vi "Rover_Planting_Commands.vi"(1 "X":dbl[](array[numeric]), 2 "Y":dbl[](array[numeric]), 3 "Seeds":bool[](array[boolean])) -> (0 "Commands":string[](array[string]), 4 "Expected":string[](array[string]), 5 "Count":i32)   [LabVIEW 2022]
doc: "Build line commands and exact acknowledgements from graph units. Does not move motors. One unit is 10 cm. Caller validates sizes and coordinate ranges."
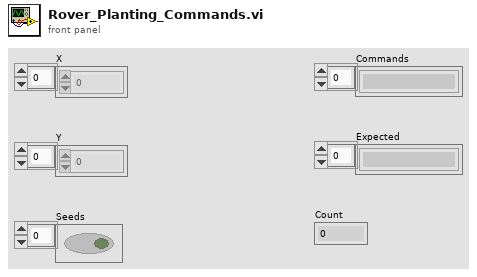
[diagram p1: front panel]
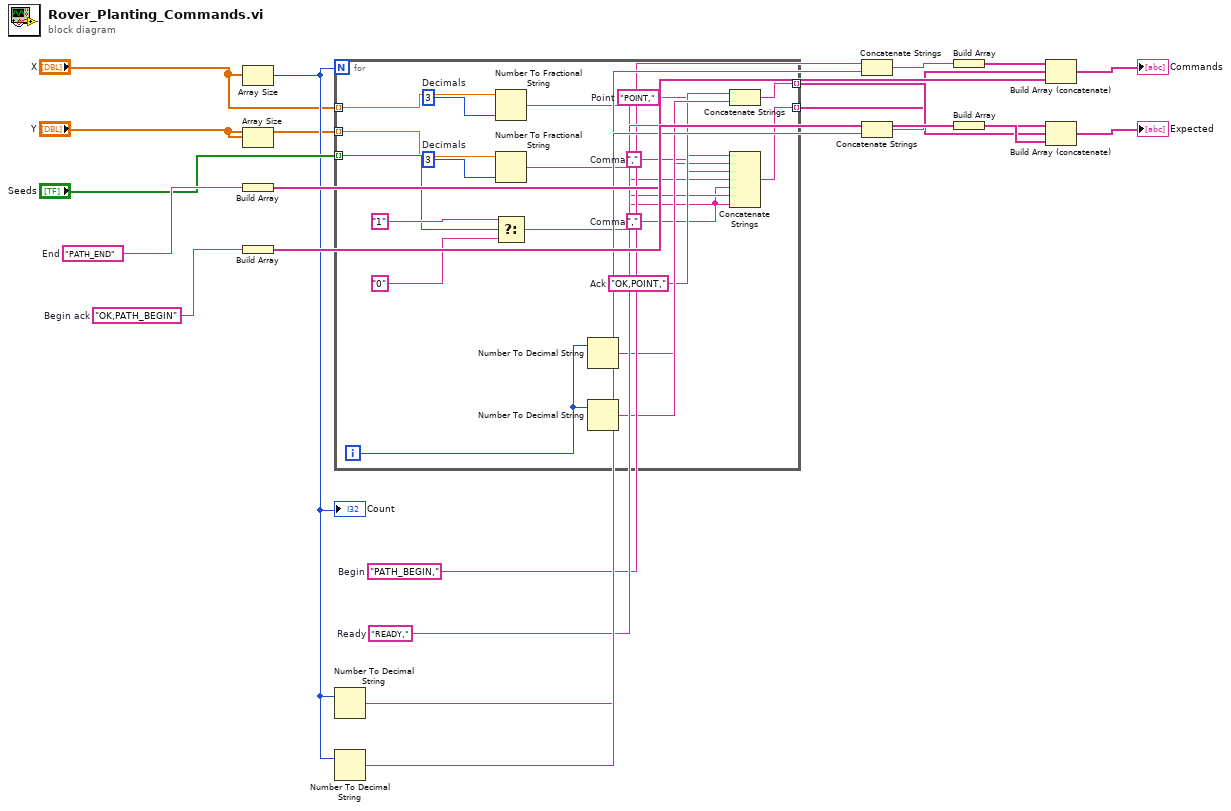
[diagram p0: block diagram]
diagram:
  w17 = "OK,PATH_BEGIN"  # Begin ack
  w14 = "PATH_END"  # End
  w10 = "READY,"  # Ready
  w7 = "PATH_BEGIN,"  # Begin
  n1 = Array Size(array="X") -> (size(s)=w3:i32)
  "Count" <- w3
  n2 = Array Size(array="Y") -> ()  [unwired: 1 out]
  n3 = Build Array(w14) -> (w15:string[])
  n4 = Build Array(w17) -> (w18:string[])
  n5 = for {
    N: w3 -> [_]
    tunnel: "X" -> [w22] mode=indexing
    tunnel: "Y" -> [w23] mode=indexing
    tunnel: "Seeds" -> [w37] mode=indexing
    tunnel: [w36] -> w5 mode=indexing
    tunnel: [w32] -> w4 mode=indexing
    i -> [w21]
    w34 = "OK,POINT,"  # Ack
    w30 = 3  # Decimals
    w29 = ","  # Comma
    w27 = 3  # Decimals
    w26 = ","  # Comma
    w24 = "POINT,"  # Point
    n6 = Number To Fractional String(number=w22, precision (6)=w27) -> (F-format string=w28:string)  [unwired: 2 out]
    n7 = Number To Fractional String(number=w23, precision (6)=w30) -> (F-format string=w31:string)  [unwired: 2 out]
    n8 = Select(t="1", s=w37, f="0") -> (s? t:f=w33:string)
    n9 = Number To Decimal String(number=w21) -> (decimal integer string=w25:string)  [unwired: 1 in]
    n10 = Number To Decimal String(number=w21) -> (decimal integer string=w35:string)  [unwired: 1 in]
    n11 = Concatenate Strings(w34, w35) -> (w36:string)
    n12 = Concatenate Strings(w24, w25, w26, w28, w29, w31, w29, w33) -> (w32:string)
  }
  n13 = Number To Decimal String(number=w3) -> (decimal integer string=w8:string)  [unwired: 1 in]
  n14 = Number To Decimal String(number=w3) -> (decimal integer string=w11:string)  [unwired: 1 in]
  n15 = Concatenate Strings(w7, w8) -> (w9:string)
  n16 = Concatenate Strings(w10, w11) -> (w12:string)
  n17 = Build Array(w9) -> (w13:string[])
  n18 = Build Array(w12) -> (w19:string[])
  n19 = Build Array (concatenate)(w13, w4, w15) -> (→"Commands":string[])
  n20 = Build Array (concatenate)(w18, w5, w19) -> (→"Expected":string[])
